vi "filter possible timestamps stored as numbers.vi"(8 "engine start":timestamp, 9 "seconds at start":dbl, 10 "SecondsSinceStart":dbl, 11 "Array in":T2(array[cluster])) -> (2 "property-to-match -> timestamp + original property":T3(c390), 3 "unmatched numerics":T1[](array[typedef]))   [LabVIEW 2020, in "nominal teststand model sequence support.lvlib"]
uses:
  nominal teststand model sequence support.lvlib
  nominal numeric result collection.ctl
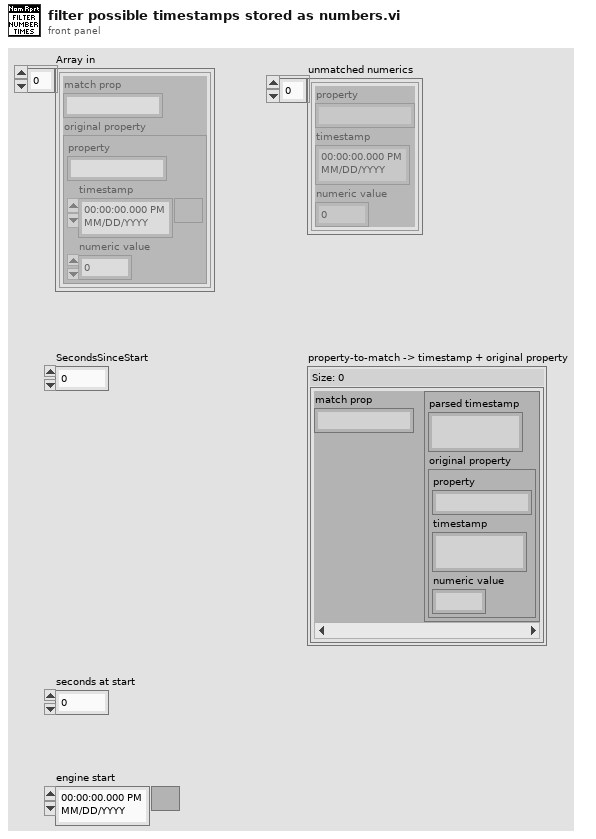
[diagram p1: front panel]
types:
  T1 = typedef "nominal teststand model sequence support.lvlib/nominal numeric result collection.ctl" = cluster{"property":string, "timestamp":timestamp, "numeric value":dbl}
  T2 = cluster{"match prop":string, "original property":T1}[]
  T3 = map{string, cluster{timestamp, "original property":T1}}
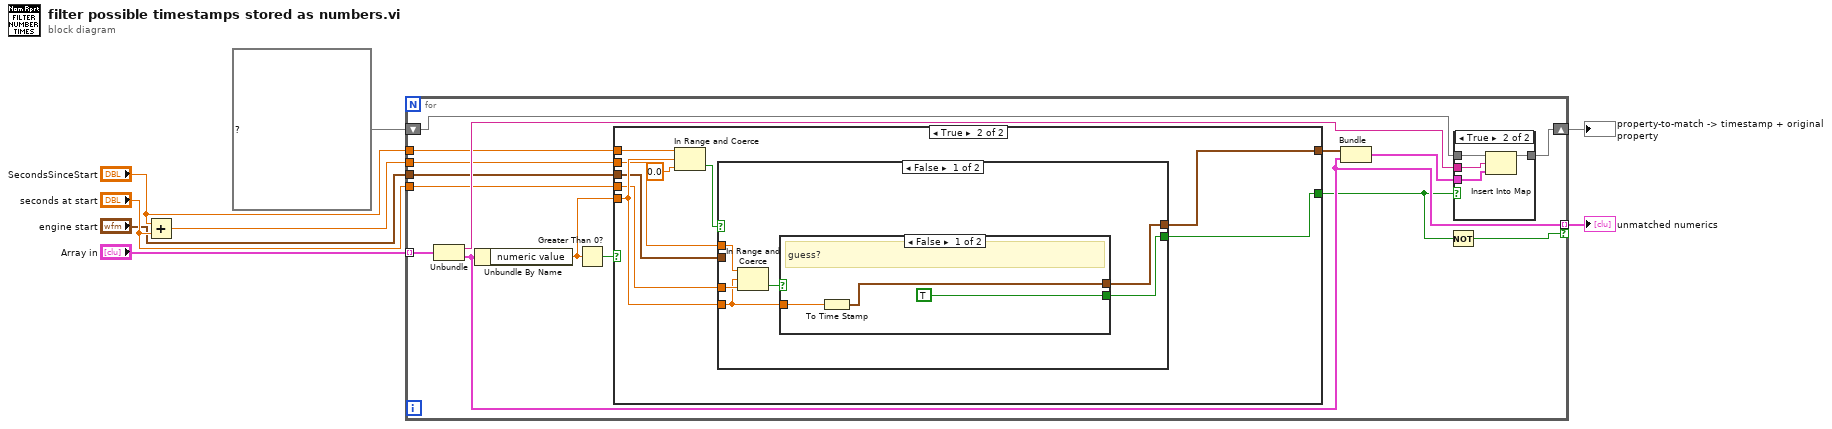
[diagram p0: block diagram]
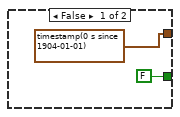
[diagram p2: hidden frame]
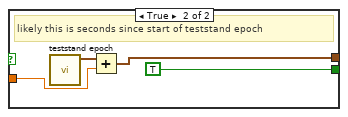
[diagram p3: hidden frame]
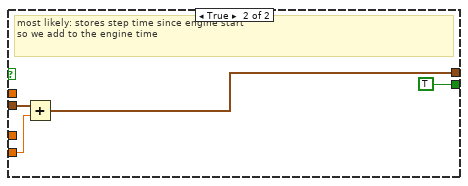
[diagram p4: hidden frame]
diagram:
  n1 = Add(x="SecondsSinceStart", y="seconds at start") -> (x+y=w8:dbl)
  n2 = for {
    tunnel: "Array in" -> [w23] mode=indexing
    tunnel: [w19] -> w3 mode=indexing if=w15
    shift-right: [w22] -> w4
    shift-left: T3 {} ("property-to-match -> timestamp + original property") -> [w21]
    tunnel: "SecondsSinceStart" -> [w17]
    tunnel: "engine start" -> [w14]
    tunnel: "seconds at start" -> [w12]
    tunnel: w8 -> [w11]
    n3 = Unbundle(w23) -> ("match prop"=w20:string, "original property"=w19:T1)
    n4 = Unbundle By Name(w19) -> ("numeric value"=w9:dbl)
    n5 = Greater Than 0?(x=w9) -> (x > 0?=w10:bool)
    n6 = case shown="True" w10 {
      tunnel: w17 -> [_ w33]
      tunnel: [FALSE w31] -> w16
      tunnel: w9 -> [_ w30]
      tunnel: w14 -> [_ w29]
      tunnel: [timestamp(0 s since 1904-01-01) w28] -> w13
      tunnel: w12 -> [_ w27]
      tunnel: w11 -> [_ w26]
      frame False {
      }
      frame True {
        n7 = In Range and Coerce(upper limit=w33, x=w30, lower limit=0.0) -> (In Range?=w32:bool)  [unwired: 1 out]
        n8 = case shown="False" w32 {
          tunnel: [w37 TRUE] -> w31
          tunnel: w30 -> [w36 w50]
          tunnel: w29 -> [_ w49]
          tunnel: [w35 w48] -> w28
          tunnel: w27 -> [w40 _]
          tunnel: w26 -> [w39 _]
          frame False {
            n9 = In Range and Coerce(upper limit=w39, x=w36, lower limit=w40) -> (In Range?=w38:bool)  [unwired: 1 out]
            n10 = case shown="False" w38 {
              tunnel: [TRUE TRUE] -> w37
              tunnel: w36 -> [w43 w45]
              tunnel: [w42 w44] -> w35
              frame False {
                # "guess?"
                n11 = To Time Stamp(1:w43) -> (0:w42:timestamp)
              }
              frame True {
                # "likely this is seconds since start of teststand epoch"
                n12 = call "teststand epoch.vi"() -> ("time stamp"=w46:timestamp)  [unwired: 11 in]
                n13 = Add(x=w46, y=w45) -> (x+y=w44:timestamp)
              }
            }
          }
          frame True {
            # "most likely: stores step time since engine start\nso we add to the engine time"
            n14 = Add(x=w49, y=w50) -> (x+y=w48:timestamp)
          }
        }
      }
    }
    n15 = Bundle(w13, "original property"=w19) -> (w18:cluster{timestamp, "original property":T1})  [unwired: 1 in]
    n16 = Not(x=w16) -> (.not. x?=w15:bool)
    n17 = case shown="True" w16 {
      tunnel: [w52 w56] -> w22
      tunnel: w21 -> [w52 w55]
      tunnel: w20 -> [_ w54]
      tunnel: w18 -> [_ w53]
      frame False {
      }
      frame True {
        n18 = Insert Into Map(map in=w55, key=w54, value=w53) -> (map out=w56:T3)  [unwired: 2 out]
      }
    }
  }
  "property-to-match -> timestamp + original property" <- w4
  "unmatched numerics" <- w3
